vi "Read Compatible Hardware Types.vi"(8 "error in (no error)":errorcluster, 11 "Measurement Test Harness in":refnum<class "Measurement Test Harness.lvclass">) -> (0 "error out":errorcluster, 2 "Compatible Hardware Types":string[](array[string]), 3 "Measurement Test Harness out":refnum<class "Measurement Test Harness.lvclass">)   [LabVIEW 2026, in "Measurement Test Harness.lvclass"]
uses:
  Measurement Test Harness.lvclass
  source/framework/Measurement Actor/Measurement.lvclass
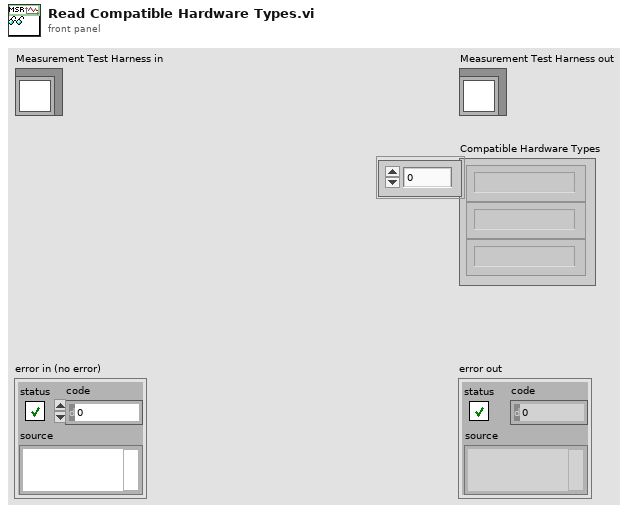
[diagram p1: front panel]
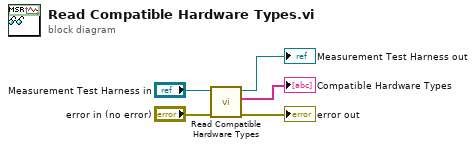
[diagram p0: block diagram]
diagram:
  n1 = call-parent "Read Compatible Hardware Types.vi"("error in (no error)"="error in (no error)", "Measurement in"="Measurement Test Harness in") -> ("error out"=→"error out":errorcluster, "Compatible Hardware Types"=→"Compatible Hardware Types":string[], "Measurement out"=→"Measurement Test Harness out":refnum<class "Measurement Test Harness.lvclass">)  [unwired: 7 in]
